vi "test--White.vi"(11 "Test Case In":refnum<class "Color to Luminance.lvclass">) -> (0 "error out":errorcluster, 3 "Test Case Out":refnum<class "Color to Luminance.lvclass">)   [LabVIEW 2021, in "Color to Luminance.lvclass"]
uses:
  Color to Luminance.lvclass
  C:/Program Files/National Instruments/LabVIEW 2026/vi.lib/Astemes/LUnit/Test Case.lvclass
  <vilib>/Astemes/LUnit/Test Case.lvclass/Test Case.ctl
  Color to Luminance.lvclass/Color to Luminance.ctl
  4993e8ee-a06a-463a-9684-69129f64d5ce.vi
  src/Material SubVIs/Material SubVIs.lvlib
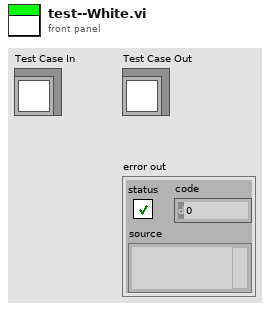
[diagram p1: front panel]
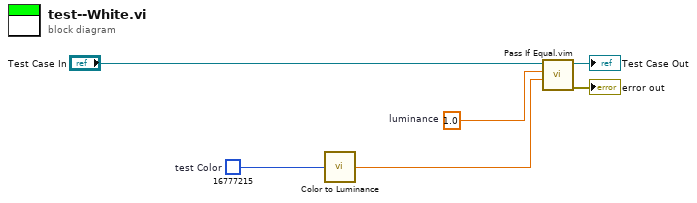
[diagram p0: block diagram]
diagram:
  w1 = 1.0  # luminance
  w3 = u32 16777215  # test Color
  n1 = call "Color to Luminance.vi"("Background Color"=w3) -> ("Luminance"=w2:dbl)
  n2 = call "Pass If Equal.vim"("Actual"=w2, "Expected"=w1, "LUnit Test Case In"="Test Case In") -> ("error out"=→"error out":errorcluster, "LUnit Test Case Out"=→"Test Case Out":refnum<class "Color to Luminance.lvclass">)  [unwired: 7 in]
